vi "Create Shared Resources.vi"(8 "error in":errorcluster, 10 "custom device ref":T1=18446744073709551615 format="%.0x", 11 "Shared Resources Factory in":refnum<class "Shared Resources Factory.lvclass">) -> (0 "error out":errorcluster, 2 "shared resources":refnum<class "Shared Resources.lvclass">, 3 "Shared Resources Factory out":refnum<class "Shared Resources Factory.lvclass">)   [LabVIEW 2020, in "AIM ARINC 429 Engine.lvlib" / "Implementation.lvlib" / "Shared Resources Factory.lvclass"]
uses:
  Shared Resources Factory.lvclass
  <vilib>/NI VeriStand/Custom Device API/Custom Device Item Ref.ctl
  Interfaces/Shared Resources/Shared Resources.lvclass
  Shared Resources/Shared Resources.lvclass
  C:/Users/nitest/Desktop/Git 2020/niveristand-aim-arinc429-custom-device/Source/Custom Device Support/Engine/Interfaces/Shared Resources/Shared Resources.lvclass
  Scripting/AIM/AIM ARINC 429 Scripting.lvlib
  <vilib>/NI VeriStand/Custom Device API/Custom Device API.lvlib
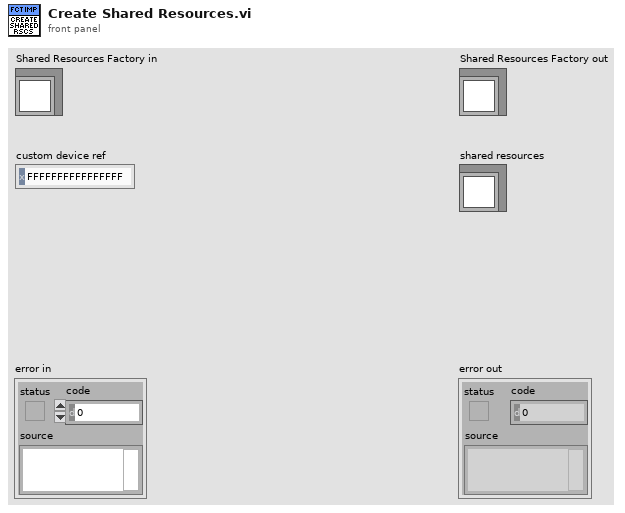
[diagram p1: front panel]
types:
  T1 = typedef "Custom Device API.lvlib/Custom Device Item Ref.ctl" = u64
  T2 = typedef "Device Parameters.ctl" = cluster{"pxi slot":u8, "coupling mode":u32}
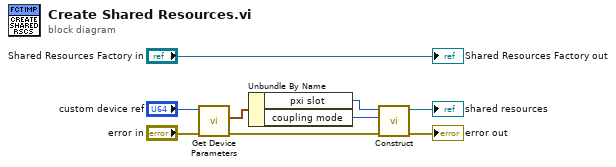
[diagram p0: block diagram]
diagram:
  n1 = call "Get Device Parameters.vi"("error in"="error in", "custom device ref"="custom device ref") -> ("error out"=w4:errorcluster, "device parameters"=w3:T2)  [unwired: 7 in, 1 out]
  n2 = Unbundle By Name(w3) -> ("pxi slot"=w2:u8, "coupling mode"=w1:u32)
  n3 = call "Construct.vi"("error in"=w4, "coupling mode"=w1, "pxi slot"=w2) -> ("error out"=→"error out":errorcluster, "Shared Resources out"=→"shared resources":refnum<class "Shared Resources.lvclass">)  [unwired: 7 in]
  "Shared Resources Factory out" <- "Shared Resources Factory in"
